vi "Iceoryx_Double_Tag.vi"() -> (3 "CIF_Iceoryx_Chn_Double.lvclass":refnum<class "CIF_Iceoryx_Chn_Double.lvclass">)   [LabVIEW 2021, in "CIF_Iceoryx_Chn_Double.lvclass"]
uses:
  CIF_Iceoryx_Chn_Double.lvclass
  CIF_Iceoryx_Chn_Double.lvclass/CIF_Iceoryx_Chn_Double.ctl
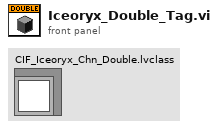
[diagram p1: front panel]
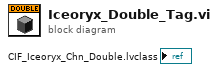
[diagram p0: block diagram]
diagram:
